vi "Add Elements to Meas Plugin UI - Multiple Converter.vi"(11 "error in":errorcluster) -> (15 "error out":errorcluster)   [LabVIEW 2021, in "Converter.lvlib"]
uses:
  Converter.lvlib
  Converter Reusables/Converter Reusables.lvlib
  Path Functions/Path Functions.lvlib
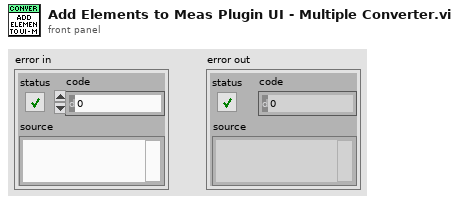
[diagram p1: front panel]
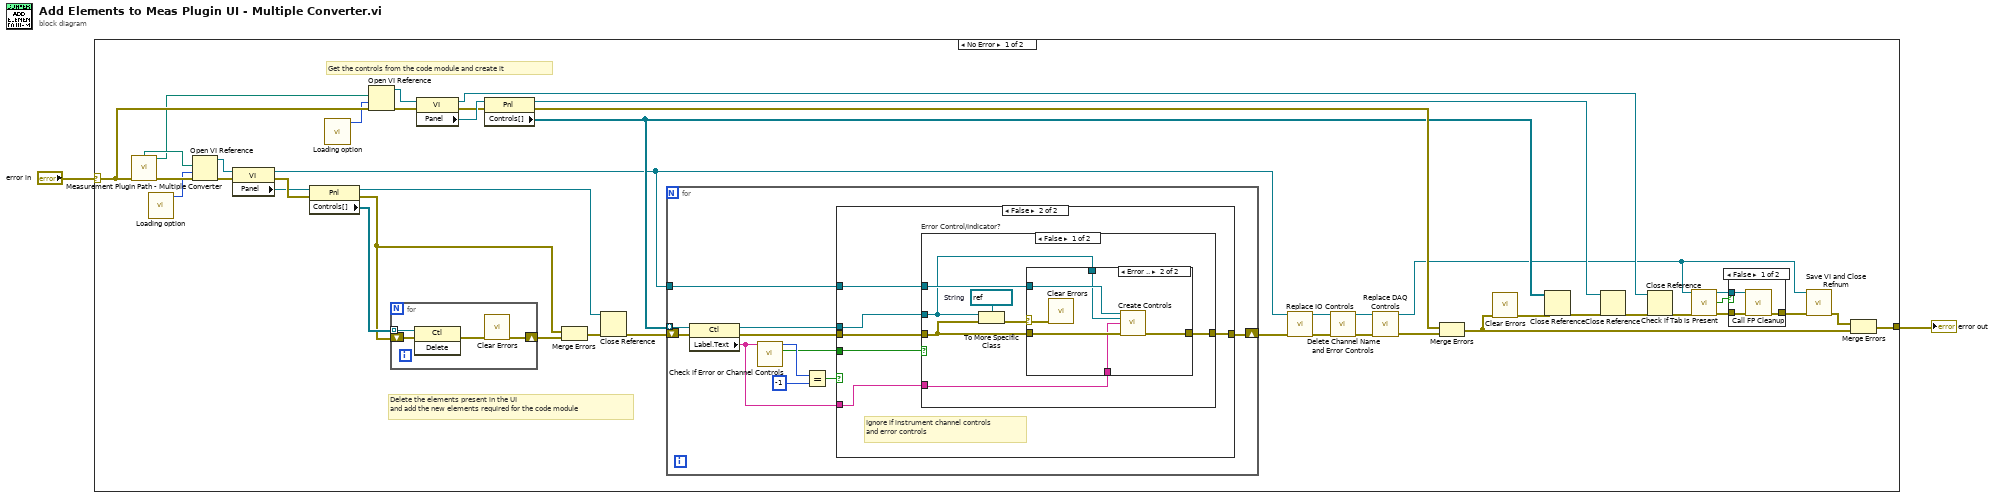
[diagram p0: block diagram]
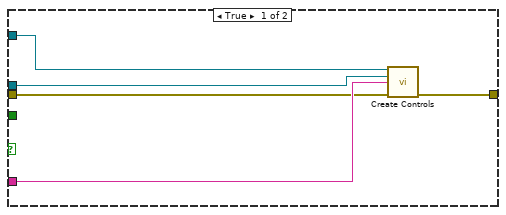
[diagram p3: hidden frame]
diagram:
  n1 = case shown="No Error" "error in" {
    selector: "error in" -> [w31 w91]
    tunnel: [w35 w91] -> w2
    frame No Error {
      # "Get the controls from the code module and create it"
      # "Delete the elements present in the UI\nand add the new elements required for the code module"
      n2 = call "Measurement Plugin Path - Multiple Converter.vi"("error in"=w31) -> ("measurement ui"=w33:path, "new code module"=w14:path, "error out"=w45:errorcluster)  [unwired: 2 in, 10 out]
      n3 = call "Loading option.vi"() -> ("options"=w4:i32)  [unwired: 11 in]
      n4 = Open VI Reference(vi path=w33, options=w4, error in (no error)=w45) -> (vi reference=w23:refnum<vi>, error out=w44:errorcluster)  [unwired: 3 in]
      n5 = property class="VI"(reference=w23, error in=w44) -> (reference out=w27:refnum<vi>, error out=w43:errorcluster, "Panel"=w29:refnum<vi>)
      n6 = property class="Pnl"(reference=w29, error in=w43) -> (reference out=w28:refnum<vi>, error out=w15:errorcluster, "Controls[]"=w42:refnum<vi>[])
      n7 = call "Loading option.vi"() -> ("options"=w3:i32)  [unwired: 11 in]
      n8 = Open VI Reference(vi path=w14, options=w3, error in (no error)=w31) -> (vi reference=w21:refnum<vi>, error out=w37:errorcluster)  [unwired: 3 in]
      n9 = for {
        tunnel: w42 -> [w90] mode=indexing
        shift-right: [w87] -> w41
        shift-left: w15 -> [w89]
        n10 = invoke class="Ctl" method="Delete"(reference=w90, error in=w89) -> (error out=w88:errorcluster)  [unwired: 1 in, 2 out]
        n11 = call <vilib>:"Clear Errors.vi"("error in (no error)"=w88) -> ("error out"=w87:errorcluster)  [unwired: 5 in, 1 out]
      }
      n12 = property class="VI"(reference=w21, error in=w37) -> (reference out=w20:refnum<vi>, error out=w36:errorcluster, "Panel"=w38:refnum<vi>)
      n13 = property class="Pnl"(reference=w38, error in=w36) -> (reference out=w19:refnum<vi>, error out=w40:errorcluster, "Controls[]"=w39:refnum<vi>[])
      n14 = Merge Errors(w15, w41) -> (w16:errorcluster)
      n15 = Close Reference(reference=w28, error in (no error)=w16) -> (error out=w30:errorcluster)
      n16 = for {
        tunnel: w27 -> [w60]
        tunnel: w39 -> [w58] mode=indexing
        shift-right: [w59] -> w26
        shift-left: w30 -> [w50]
        n17 = property class="Ctl"(reference=w58, error in=w50) -> (reference out=w56:refnum<vi>, error out=w55:errorcluster, "Label.Text"=w57:string)
        n18 = call "Check if Error or Channel Controls.vi"("label.text"=w57) -> ("error?"=w51:bool, "offset past match"=w54:i32)  [unwired: 9 in]
        n19 = Equal?(x=w54, y=-1) -> (x = y?=w52:bool)
        n20 = case shown="False" w52 {
          tunnel: w60 -> [w65 w68]
          tunnel: [w64 w66] -> w59
          tunnel: w56 -> [w62 w71]
          tunnel: w55 -> [w61 w70]
          tunnel: w57 -> [w63 w67]
          tunnel: w51 -> [_ w69]
          frame True {
            n21 = call "Create Controls.vi"("vi in"=w65, "ctl refnum"=w62, "control label"=w63, "error in"=w61) -> ("error out"=w64:errorcluster)  [unwired: 11 in]
          }
          frame False {
            # "Ignore if instrument channel controls\nand error controls"
            n22 = case "Error Control/Indicator?" shown="False" w69 {
              tunnel: w71 -> [w74 _]
              tunnel: w70 -> [w77 w86]
              tunnel: w68 -> [w75 _]
              tunnel: w67 -> [w73 _]
              tunnel: [w72 w86] -> w66
              frame False {
                w78 = refnum<vi> refnum  # String
                n23 = To More Specific Class(target class=w78, reference=w74, error in=w77) -> (error out=w76:errorcluster)  [unwired: 1 out]
                n24 = case shown="Error .." w76 {
                  selector: w76 -> [_ w80]
                  tunnel: w77 -> [w79 w85]
                  tunnel: w75 -> [_ w84]
                  tunnel: w74 -> [_ w83]
                  tunnel: w73 -> [_ w82]
                  tunnel: [w79 w81] -> w72
                  frame No Error {
                  }
                  frame Error {
                    n25 = call <vilib>:"Clear Errors.vi"("error in (no error)"=w80) -> ()  [unwired: 5 in, 2 out]
                    n26 = call "Create Controls.vi"("vi in"=w84, "ctl refnum"=w83, "control label"=w82, "error in"=w85) -> ("error out"=w81:errorcluster)  [unwired: 11 in]
                  }
                }
              }
              frame True {
              }
            }
          }
        }
      }
      n27 = call "Replace IO Controls.vi"("vi in"=w27, "error in"=w26) -> ("vi out"=w25:refnum<vi>, "error out"=w24:errorcluster)  [unwired: 12 in]
      n28 = call "Delete Channel Name and Error Controls.vi"("vi in"=w25, "error in"=w24) -> ("vi out"=w9:refnum<vi>, "error out"=w6:errorcluster)  [unwired: 12 in]
      n29 = call "Replace DAQ Controls.vi"("vi in"=w9, "error in"=w6) -> ("vi out"=w8:refnum<vi>, "error out"=w7:errorcluster)  [unwired: 12 in]
      n30 = Merge Errors(w40, w7) -> (w5:errorcluster)
      n31 = call <vilib>:"Clear Errors.vi"("error in (no error)"=w5) -> ("error out"=w34:errorcluster)  [unwired: 5 in, 1 out]
      n32 = Close Reference(reference=w39, error in (no error)=w34) -> (error out=w17:errorcluster)
      n33 = Close Reference(reference=w19, error in (no error)=w17) -> (error out=w18:errorcluster)
      n34 = Close Reference(reference=w20, error in (no error)=w18) -> (error out=w12:errorcluster)
      n35 = call "Check if Tab is Present.vi"("vi in"=w8, "error in"=w12) -> ("vi out"=w13:refnum<vi>, "tab present?"=w10:bool, "error out"=w11:errorcluster)  [unwired: 11 in]
      n36 = case shown="False" w10 {
        tunnel: [w48 w49] -> w22
        tunnel: w13 -> [w47 _]
        tunnel: w11 -> [w46 w49]
        frame False {
          n37 = call "Call FP Cleanup.vi"("vi"=w47, "error in"=w46) -> ("error out"=w48:errorcluster)  [unwired: 13 in]
        }
        frame True {
        }
      }
      n38 = call "Save VI and Close Refnum.vi"("vi refnum"=w8, "error in"=w22) -> ("error out"=w32:errorcluster)  [unwired: 13 in]
      n39 = Merge Errors(w32, w5) -> (w35:errorcluster)
    }
    frame Error {
    }
  }
  "error out" <- w2
